vi "query BandWidth.vi"(8 "error in (no error)":errorcluster, 9 "LTE Channel Type":T2, 11 "LTE in":refnum<class "LTE.lvclass">) -> (0 "error out":errorcluster, 2 "BandWidth":T1, 3 "LTE out":refnum<class "LTE.lvclass">)   [LabVIEW 2023, in "ANRITSU Call Box.lvlib" / "LTE.lvclass"]
uses:
  LTE.lvclass
  Type Definition/LTE Channel Type.ctl
  Type Definition/LTE Supported BandWidth.ctl
  LTE.lvclass/LTE.ctl
  <vilib>/Utility/error.llb/Trim Whitespace One-Sided.vi
  ANRITSU Call Box.lvlib
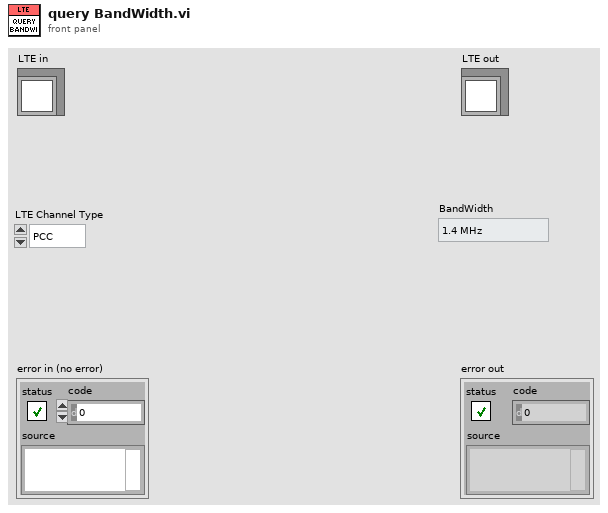
[diagram p1: front panel]
types:
  T1 = typedef "ANRITSU Call Box.lvlib/LTE Supported BandWidth.ctl" = enum16{"1.4 MHz", "3 MHz", "5 MHz", "10 MHz", "15 MHz", "20 MHz"}
  T2 = typedef "ANRITSU Call Box.lvlib/LTE Channel Type.ctl" = enum16{"PCC", "SCC1", "SCC2", "SCC3"}
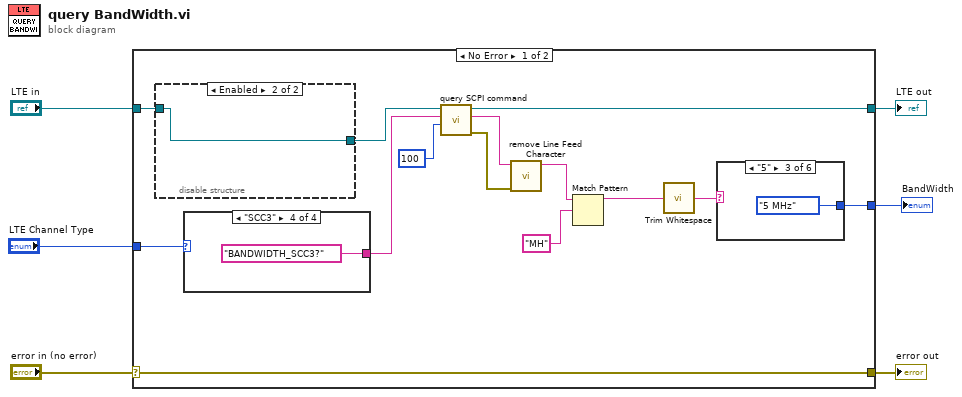
[diagram p0: block diagram]
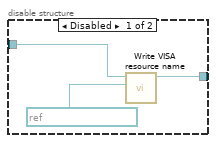
[diagram p2: hidden frame]
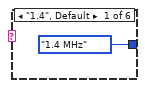
[diagram p3: hidden frame]
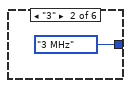
[diagram p4: hidden frame]
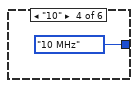
[diagram p5: hidden frame]
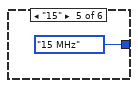
[diagram p6: hidden frame]
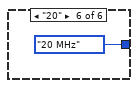
[diagram p7: hidden frame]
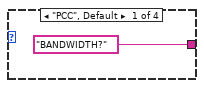
[diagram p8: hidden frame]
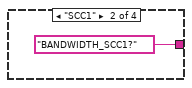
[diagram p9: hidden frame]
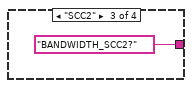
[diagram p10: hidden frame]
diagram:
  n1 = case shown="No Error" "error in (no error)" {
    selector: "error in (no error)" -> [w20 w36]
    tunnel: [w20 w36] -> w5
    tunnel: [w11 w35] -> w3
    tunnel: "LTE in" -> [w8 w35]
    tunnel: "LTE Channel Type" -> [w19 _]
    tunnel: [w9 _] -> w1
    frame No Error {
      n2 = disable-structure shown="Enabled" {
        disable-tunnel: w8 -> [w23 w24]
        disable-tunnel: [w21 w24] -> w7
        frame Disabled {
          n3 = call "Write VISA resource name.vi"("VISA resource name"=refnum<visa-resource-name> "GPIB0::1::INSTR", "LTE in"=w23) -> ("LTE out"=w21:refnum<class "LTE.lvclass">)  [unwired: 8 in, 1 out]
        }
        frame Enabled {
        }
      }
      n4 = case shown="\"SCC3\"" w19 {
        tunnel: ["BANDWIDTH?" ("string") "BANDWIDTH_SCC1?" ("string") "BANDWIDTH_SCC2?" ("string") "BANDWIDTH_SCC3?" ("string")] -> w18
        frame "PCC", Default {
        }
        frame "SCC1" {
        }
        frame "SCC2" {
        }
        frame "SCC3" {
        }
      }
      n5 = call "query SCPI command.vi"("Read Buffer Length"=u32 100, "SCPI Command"=w18, "LTE in"=w7) -> ("error out"=w15:errorcluster, "Read Buffer String"=w16:string, "LTE out"=w11:refnum<class "LTE.lvclass">)  [unwired: 6 in]
      n6 = call "remove Line Feed Character.vi"("error in"=w15, "Query String"=w16) -> ("Line Feed Removed String"=w14:string)  [unwired: 8 in, 1 out]
      n7 = Match Pattern(string=w14, regular expression="MH") -> (before substring=w12:string)  [unwired: 1 in, 3 out]
      n8 = call <vilib>:"Trim Whitespace.vi"("string"=w12) -> ("trimmed string"=w10:string)  [unwired: 1 in]
      n9 = case shown="\"5\"" w10 {
        tunnel: [LTE_Supported_BandWidth."1.4 MHz" ("BandWidth 2") LTE_Supported_BandWidth."3 MHz" ("BandWidth 2") LTE_Supported_BandWidth."5 MHz" ("BandWidth 2") LTE_Supported_BandWidth."10 MHz" ("BandWidth 2") LTE_Supported_BandWidth."15 MHz" ("BandWidth 2") LTE_Supported_BandWidth."20 MHz" ("BandWidth 2")] -> w9
        frame "1.4", Default {
        }
        frame "3" {
        }
        frame "5" {
        }
        frame "10" {
        }
        frame "15" {
        }
        frame "20" {
        }
      }
    }
    frame Error {
    }
  }
  "error out" <- w5
  "LTE out" <- w3
  "BandWidth" <- w1
